vi "Init_Comm.vi"(8 "error in":errorcluster) -> (0 "error out":errorcluster, 3 "rt fifo ref out":refnum<k33>)   [LabVIEW 2025]
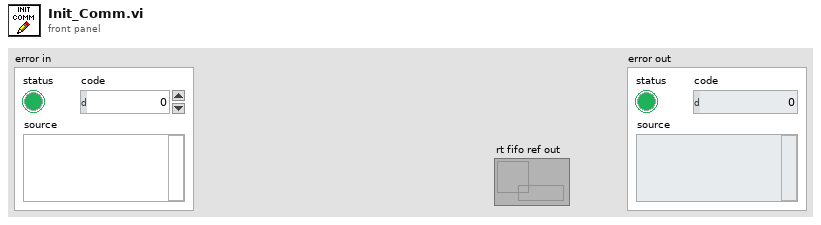
[diagram p1: front panel]
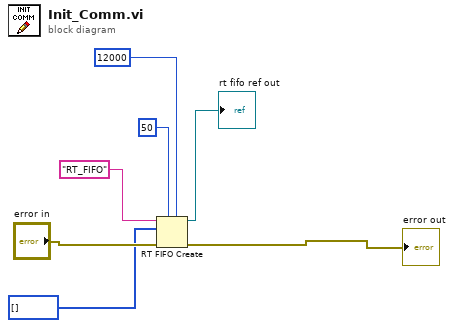
[diagram p0: block diagram]
diagram:
  n1 = RT FIFO Create(0:"RT_FIFO" ("name (unnamed)"), 1:i16[] [], 3:"error in", 4:u32 50 ("size (10)"), 6:u32 12000 ("elements in array (1)")) -> (8:→"rt fifo ref out":refnum<k33>, 11:→"error out":errorcluster)  [unwired: 3 in, 1 out]
